vi "Read Write.vi"(8 "error in (no error)":errorcluster, 9 "RW":T1=enum."Write", 10 "Buffer In":u8[](array[numeric])=[0, 255, 2, 0, 0, 0, 0, 0, 0] format="%.0x", 11 "HID Handle":i64) -> (0 "error out":errorcluster, 2 "Buffer Out":u8[](array[numeric]) format="%.0x")   [LabVIEW 2021, in "USB Relay Control.lvlib"]
uses:
  USB Relay Control.lvlib
  typedef/Read Write.ctl
  hid.dll
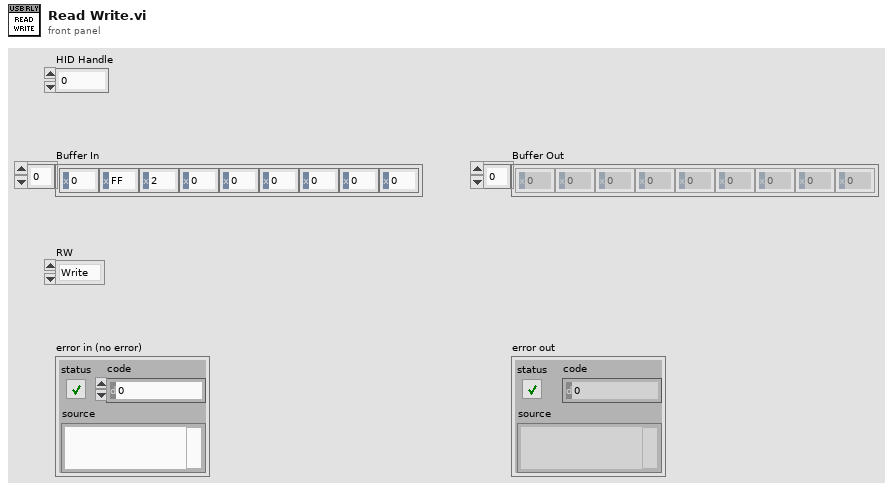
[diagram p1: front panel]
types:
  T1 = typedef "USB Relay Control.lvlib/Read Write.ctl" = enum8{"Read", "Write"}
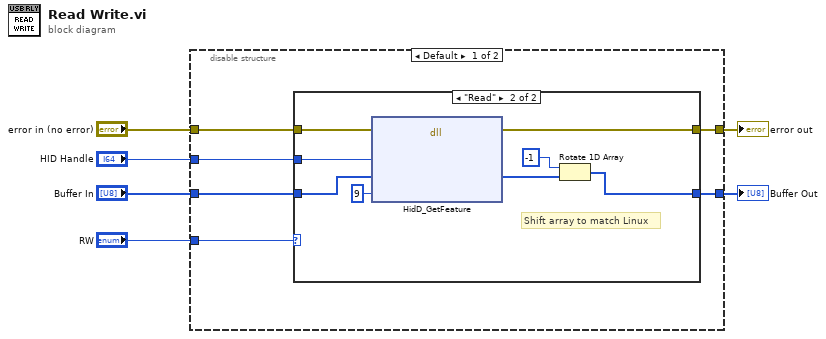
[diagram p0: block diagram]
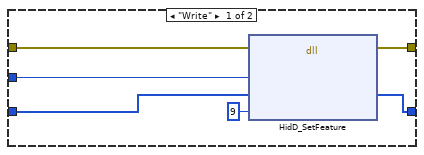
[diagram p2: hidden frame]
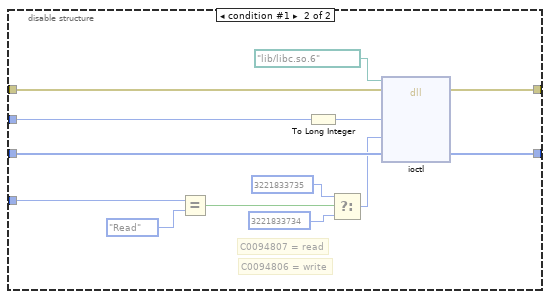
[diagram p3: hidden frame]
diagram:
  n1 = disable-structure shown="Default" {
    disable-tunnel: "Buffer In" -> [w12 w39]
    disable-tunnel: [w11 w38] -> w5
    disable-tunnel: "error in (no error)" -> [w10 w37]
    disable-tunnel: "HID Handle" -> [w8 w36]
    disable-tunnel: [w9 w35] -> w2
    disable-tunnel: "RW" -> [w7 w31]
    frame condition #0 (active) {
      n2 = case shown="\"Read\"" w7 {
        tunnel: w12 -> [w18 w26]
        tunnel: [w17 w19] -> w11
        tunnel: w10 -> [w16 w25]
        tunnel: [w15 w24] -> w9
        tunnel: w8 -> [w14 w23]
        frame "Write" {
          n3 = dll-call lib="hid.dll" fn="HidD_SetFeature"(error in=w16, "HidDeiviceObject"=w14, "ReportBuffer"=w18, "ReportBufferLength"=u32 9) -> (error out=w15:errorcluster, "ReportBuffer"=w17:u8[])  [unwired: 5 in, 1 out]
        }
        frame "Read" {
          # "Shift array to match Linux"
          n4 = dll-call lib="hid.dll" fn="HidD_GetFeature"(error in=w25, "HidDeiviceObject"=w23, "ReportBuffer"=w26, "ReportBufferLength"=u32 9) -> (error out=w24:errorcluster, "ReportBuffer"=w21:u8[])  [unwired: 5 in, 1 out]
          n5 = Rotate 1D Array(1:w21, 2:-1 ("n")) -> (0:w19:u8[])
        }
      }
    }
    frame condition #1 {
      # "C0094806 = write"
      # "C0094807 = read"
      n6 = Equal?(x=w31, y=Read_Write."Read") -> (x = y?=w29:bool)
      n7 = To Long Integer(number=w36) -> (32bit integer=w27:i32)
      n8 = Select(t=u64 3221833735 ("request"), s=w29, f=u64 3221833734 ("request")) -> (s? t:f=w28:u64)
      n9 = dll-call lib="lib/libc.so.6" fn="ioctl"(path in=path "/lib/libc.so.6" ("librt path"), error in=w37, "fd"=w27, "request"=w28, "buf"=w39) -> (error out=w35:errorcluster, "buf"=w38:u8[])  [unwired: 4 in, 1 out]
    }
  }
  "error out" <- w2
  "Buffer Out" <- w5
